vi "update.name.vi"(8 "error in (no error)":errorcluster, 10 "Title":string, 11 "Run in":refnum<class "Run.lvclass">) -> (0 "error out":errorcluster, 3 "Run out":refnum<class "Run.lvclass">)   [LabVIEW 2020, in "Run.lvclass"]
uses:
  Run.lvclass
  Nominal Client/Nominal Client.lvclass
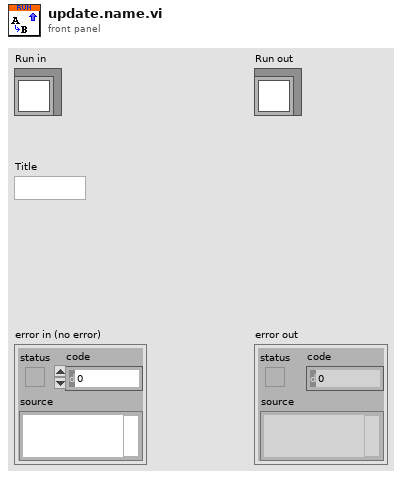
[diagram p1: front panel]
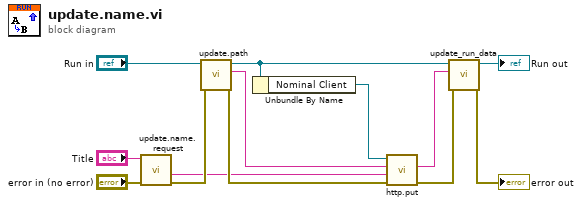
[diagram p0: block diagram]
diagram:
  n1 = call "update.name.request.vi"("error in"="error in (no error)", "Title"="Title") -> ("error out"=w4:errorcluster, "Request"=w2:string)  [unwired: 8 in]
  n2 = call "update.path.vi"("error in"=w4, "Run"="Run in") -> ("error out"=w3:errorcluster, "path"=w10:string, "Run Out"=w9:refnum<class "Run.lvclass">)  [unwired: 7 in]
  n3 = Unbundle By Name(w9) -> ("Nominal Client"=w11:refnum<class "Nominal Client.lvclass">)
  n4 = call "http.put.vi"("error in"=w3, "Body"=w2, "Path"=w10, "Nominal Client in"=w11) -> ("error out"=w8:errorcluster, "Response"=w7:string)  [unwired: 5 in, 1 out]
  n5 = call "update_run_data.vi"("error in"=w8, "Run JSON"=w7, "Run in"=w9) -> ("error out"=→"error out":errorcluster, "Run out"=→"Run out":refnum<class "Run.lvclass">)  [unwired: 7 in]
